vi "user32 GetKeyboardState.vi"(11 "error in":errorcluster) -> (4 "key state":u8[](array[numeric]), 6 "return value":i32, 15 "error out":errorcluster)   [LabVIEW 2020, in "RemoteVI.lvlib"]
doc: "Reads the key state of the CALLING thread through user32.dll GetKeyboardState (stdcall, called in LabVIEW's UI thread): one byte per virtual-key code, bit 0x80 set while the key is down, bit 0x01 the toggle state. Windows keeps this state per thread and updates it only when the thread retrieves input from the real input queue - posted messages leave it alone. Running in the UI thread, this is the state LabVIEW's panels read for the modifier keys (GetKeyState). return value is the Win32 BOOL: non-zero on success, 0 on failure. When error in carries an error the DLL is not called. Generated by scripts\\Build Win32 Wrappers.vi - do not edit by hand, rebuild it."
uses:
  RemoteVI.lvlib
  user32.dll
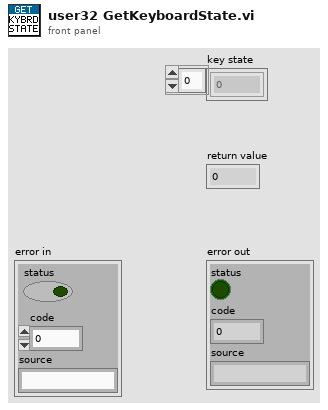
[diagram p1: front panel]
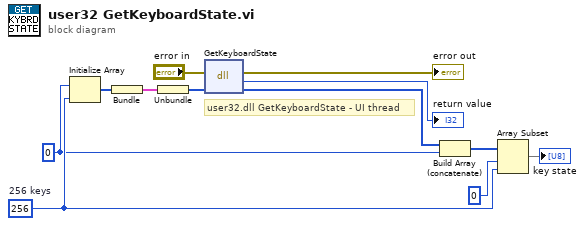
[diagram p0: block diagram]
diagram:
  w8 = 256  # 256 keys
  w7 = u8 0
  # "user32.dll GetKeyboardState - UI thread"
  n1 = Initialize Array(w7, w8) -> (w10:u8[])
  n2 = Bundle(w10) -> (w11:cluster{u8[]})  [unwired: 1 in]
  n3 = Unbundle(w11) -> (w2:u8[])
  n4 = dll-call lib="user32.dll" fn="GetKeyboardState"(error in="error in", "lpKeyState"=w2) -> (error out=→"error out":errorcluster, →"return value":i32, "lpKeyState"=w1:u8[])  [unwired: 2 in, 1 out]
  n5 = Build Array (concatenate)(w1, w7) -> (w12:u8[])
  n6 = Array Subset(array=w12, index=0, length=w8) -> (→"key state":u8[])
